vi "New F-String Formatter.vi"(6 "include namespaces? (F)":bool, 8 "length (-1: Full)":i32=-1, 9 "# of callers (-1: All)":i32=-1, 10 "delimiter (\" > \")":string=" > ", 11 "format string (\"%T | %L | %M\")":string="%^<%Y-%m-%dT%H:%M:%S%3uZ>T | %-8L | %M") -> (3 "new f-string formatter":refnum<class "Format String.lvclass">)   [LabVIEW 2018, in "GLog.lvlib" / "Format String.lvclass"]
doc: "Creates a new Formatter which formats a log record into a string based on the Format String defined by the user. \n\nAll standard Format Specifiers are supported, included the following custom ones:\n- %M formats the log records Message field. It supports the same modifiers as the standard %s specifier.\n- %L formats the log record's Log Level field. It supports the same modifiers as the standard %s specifier.\n- %C formats the log record's Call Chain field. Fine-grained control of the Call Chain formatting is handled with the configuration arguments to this VI rather than modifiers.\n- %{fieldname}s will format the log record's Data field, using the provided fieldname as the value to format. The format specifier does not have to be \"s\", any of the default specifiers are supported, however the datatype of the fieldname must be appropriate for the format specifier used after the curly braces. This specifier also supports the same modifiers that are supported by the specifier used in the string. If the data field of the log record contains a cluster, dot notation (field.subfield.subsubfield) can be used to specify the exact value to be formatted. \".\" and \"\\\" characters can be escaped with a preceding \"\\\" character."
uses:
  Format String.lvclass
  Format String.lvclass/Format String.ctl
panel:
  # "Connector Pane"
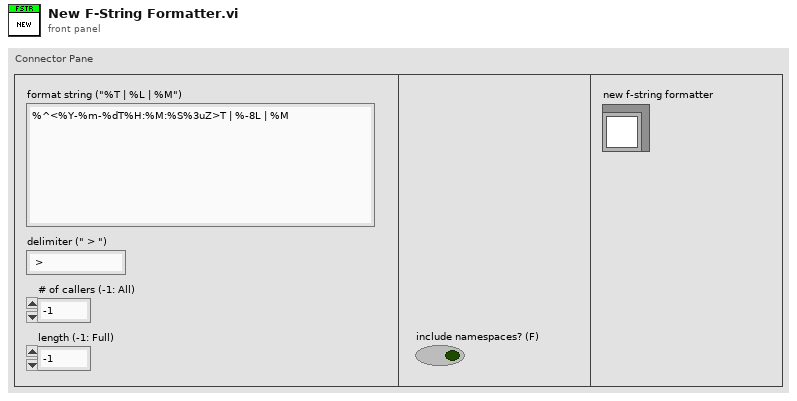
[diagram p1: front panel]
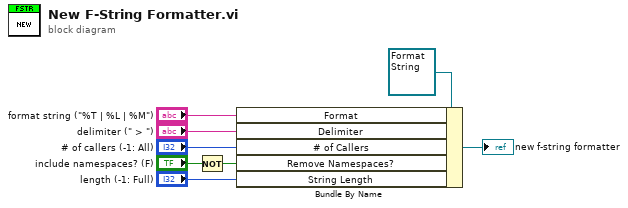
[diagram p0: block diagram]
diagram:
  n1 = Not(x="include namespaces? (F)") -> (.not. x?=w1:bool)
  n2 = Bundle By Name(cluster=refnum<class "Format String.lvclass"> refnum ("new f-string formatter"), "Format"="format string (\"%T | %L | %M\")", "Delimiter"="delimiter (\" > \")", "# of Callers"="# of callers (-1: All)", "Remove Namespaces?"=w1, "String Length"="length (-1: Full)") -> (→"new f-string formatter":refnum<class "Format String.lvclass">)
